vi "Create Empty.vi"(8 "error in (no error)":errorcluster) -> (0 "error out":errorcluster, 3 "Empty Buffer":refnum<class "Buffer.lvclass">)   [LabVIEW 2020, in "Buffer.lvclass"]
doc: "Create an empty buffer which can be passed to the Camera to store image data into."
uses:
  Buffer.lvclass
  Buffer.lvclass/Buffer.ctl
  bin/gindustrialcam_32-1.dll
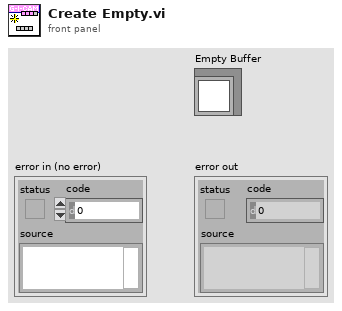
[diagram p1: front panel]
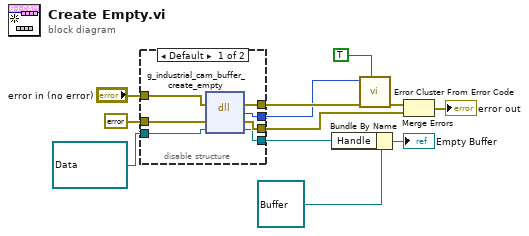
[diagram p0: block diagram]
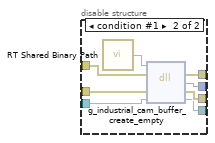
[diagram p2: hidden frame]
diagram:
  n1 = disable-structure shown="Default" {
    disable-tunnel: [w19 w27] -> w10
    disable-tunnel: [w18 w26] -> w9
    disable-tunnel: [w17 w25] -> w7
    disable-tunnel: errorcluster {"status"=FALSE, "code"=0, "source"=""} ("error constant") -> [w16 w24]
    disable-tunnel: "error in (no error)" -> [w15 w23]
    disable-tunnel: refnum<data-value> refnum ("Handle") -> [w14 w22]
    disable-tunnel: [w13 w21] -> w1
    frame condition #0 (active) {
      n2 = dll-call lib="C:/serenial/lib/g-industrial-camera/LabVIEW/g_industrial_cam/bin/gindustrialcam_*-1.*" fn="g_industrial_cam_buffer_create_empty"(error in=w15, "err"=w16, "edvr"=w14) -> (error out=w19:errorcluster, "Mg_Error"=w18:i32, "err"=w17:errorcluster, "edvr"=w13:refnum<data-value>)  [unwired: 2 in, 1 out]
    }
    frame condition #1 {
      n3 = call "RT Shared Binary Path.vi"() -> ("Path"=w20:path)
      n4 = dll-call lib="C:/serenial/lib/g-industrial-camera/LabVIEW/g_industrial_cam/bin/gindustrialcam_*-1.*" fn="g_industrial_cam_buffer_create_empty"(path in=w20, error in=w23, "err"=w24, "edvr"=w22) -> (error out=w27:errorcluster, "Mg_Error"=w26:i32, "err"=w25:errorcluster, "edvr"=w21:refnum<data-value>)  [unwired: 1 in, 1 out]
    }
  }
  n5 = Bundle By Name(cluster=refnum<class "Buffer.lvclass"> refnum ("Buffer in"), "Handle"=w1) -> (→"Empty Buffer":refnum<class "Buffer.lvclass">)
  n6 = call <vilib>:"Error Cluster From Error Code.vi"("show call chain? (False)"=TRUE, "error in (no error)"=w10, "error code (0)"=w9) -> ("error out"=w8:errorcluster)  [unwired: 6 in]
  n7 = Merge Errors(w8, w7) -> (→"error out":errorcluster)
